vi "Run All.vi"(8 "Error In":errorcluster) -> (0 "Error Out":errorcluster)   [LabVIEW 2018, in "Tests.lvlib"]
uses:
  Tests.lvlib
  Version/Version.lvlib
  Writer/Writer.lvlib
  <vilib>/addons/_JKI Toolkits/Caraya/classes/Test/Test.lvclass
  Status/Status.lvlib
  To Msgpack/To Msgpack.lvlib
  Reader/Reader.lvlib
  From Msgpack/From Msgpack.lvlib
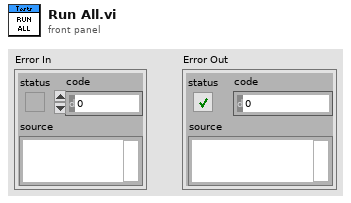
[diagram p1: front panel]
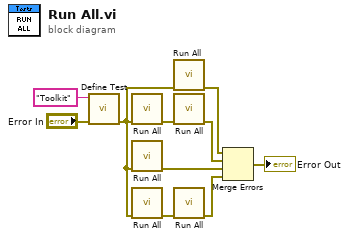
[diagram p0: block diagram]
diagram:
  n1 = call <vilib>:"Define Test.vi"("error in (no error)"="Error In", "Label (VI Title)"="Toolkit") -> ("error out"=w3:errorcluster)  [unwired: 9 in]
  n2 = call "Run All.vi"("Error In"=w3) -> ("Error Out"=w5:errorcluster)  [unwired: 10 in]
  n3 = call "Run All.vi"("Error In"=w3) -> ("Error Out"=w6:errorcluster)  [unwired: 10 in]
  n4 = call "Run All.vi"("Error In"=w3) -> ("Error Out"=w2:errorcluster)  [unwired: 10 in]
  n5 = call "Run All.vi"("Error In"=w3) -> ("Error Out"=w10:errorcluster)  [unwired: 10 in]
  n6 = call "Run All.vi"("Error In"=w5) -> ("Error Out"=w4:errorcluster)  [unwired: 10 in]
  n7 = call "Run All.vi"("Error In"=w2) -> ("Error Out"=w1:errorcluster)  [unwired: 10 in]
  n8 = Merge Errors(w10, w4, w6, w1) -> (→"Error Out":errorcluster)
